vi "Search Help.vi"(8 "error in (no error)":errorcluster, 10 "search term":string) -> (0 "error out":errorcluster)   [LabVIEW 2023, in "GettingStartedWindow.lvlib"]
uses:
  <resource>/modes/FRC/GettingStartedWindow.lvlib
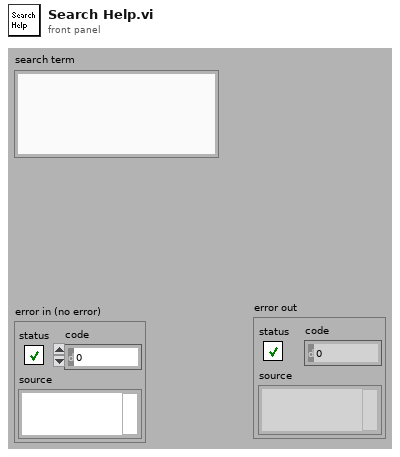
[diagram p1: front panel]
types:
  T1 = cluster{"Keyword":bool, "Full Text":bool, "Any Words":bool, "All Words":bool}
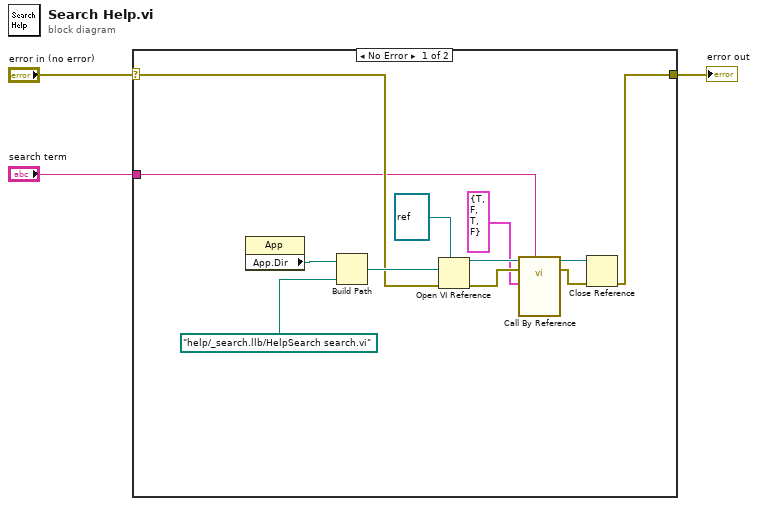
[diagram p0: block diagram]
diagram:
  n1 = case shown="No Error" "error in (no error)" {
    selector: "error in (no error)" -> [w8 w16]
    tunnel: [w5 w16] -> w2
    tunnel: "search term" -> [w4 _]
    frame No Error {
      n2 = property class="App"() -> ("App.Dir"=w15:path)  [unwired: 2 in, 2 out]
      n3 = Build Path(base path=w15, name or relative path=path "help/_search.llb/HelpSearch search.vi") -> (appended path=w13:path)
      n4 = Open VI Reference(type specifier VI Refnum (for type only)=refnum<vi> refnum, vi path=w13, error in (no error)=w8) -> (vi reference=w12:refnum<vi>, error out=w11:errorcluster)  [unwired: 3 in]
      n5 = call-by-ref "?"(reference=w12, error in=w11, "Search words"=w4, "radio buttons"=T1 {"Keyword"=TRUE, "Full Text"=FALSE, "Any Words"=TRUE, "All Words"=FALSE}) -> (reference out=w7:refnum<vi>, error out=w6:errorcluster)  [unwired: 9 in, 1 out]
      n6 = Close Reference(reference=w7, error in (no error)=w6) -> (error out=w5:errorcluster)
    }
    frame Error {
    }
  }
  "error out" <- w2
